vi "AssertControlInVisible_Tests.vi"(8 "error in":errorcluster) -> (0 "error out":errorcluster)   [LabVIEW 2016, in "DronaTest.lvlib"]
uses:
  DronaTest.lvlib
  APIs/Stimulus/ControlValue/ValueSignalByPathString.vi
  APIs/Assert/AssertControlProperty/AssertControlVisible/AssertInvisible.vi
  Drona.lvlib
  APIs/Stimulus/ControlValue/ControlValue.lvlib
  <vilib>/addons/_JKI Toolkits/Caraya/classes/Test/Test.lvclass
  APIs/Assert/AssertControlProperty/AssertControlVisible/AssertControlVisible.lvlib
  <vilib>/addons/_JKI Toolkits/Caraya/classes/Assert/Assert.lvclass
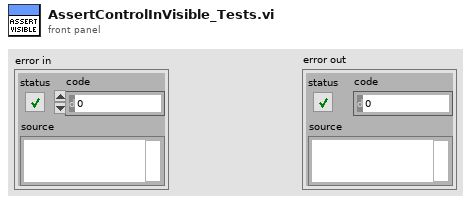
[diagram p1: front panel]
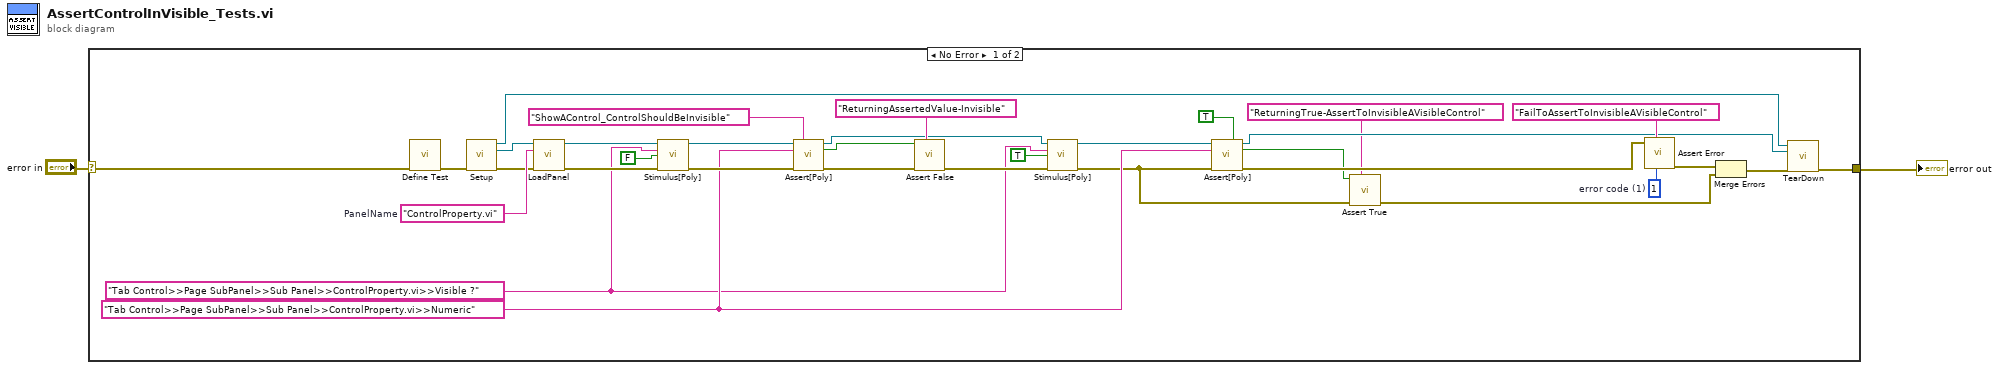
[diagram p0: block diagram]
diagram:
  n1 = case shown="No Error" "error in" {
    selector: "error in" -> [w35 w36]
    tunnel: [w25 w36] -> w1
    frame No Error {
      w13 = 1  # error code (1)
      w15 = "Tab Control>>Page SubPanel>>Sub Panel>>ControlProperty.vi>>Numeric" ("Control Path")
      w8 = "Tab Control>>Page SubPanel>>Sub Panel>>ControlProperty.vi>>Visible ?" ("Control Path")
      w34 = "ControlProperty.vi"  # PanelName
      n2 = call <vilib>:"Define Test.vi"("error in (no error)"=w35) -> ("error out"=w28:errorcluster)  [unwired: 9 in, 1 out]
      n3 = call "Setup.vi"("error in"=w28) -> ("Application Ref"=w24:refnum<vi>, "VI out"=w29:refnum<vi>, "error out"=w30:errorcluster)  [unwired: 12 in]
      n4 = call "LoadPanel.vi"("VI in"=w29, "Item Name"=w34, "error in"=w30) -> ("VI out"=w21:refnum<vi>, "error out"=w31:errorcluster)  [unwired: 11 in]
      n5 = call-poly "Stimulus[Poly].vi"("VI Reference In"=w21, "Control Path"=w8, "Value (Signaling)"=FALSE, "error in"=w31) -> ("VI Reference Out"=w33:refnum<vi>, "error out"=w23:errorcluster)  [unwired: 10 in]
      n6 = call-poly "Assert[Poly].vi"("VI Reference In"=w33, "Label"="ShowAControl_ControlShouldBeInvisible" ("string"), "Control Path"=w15, "Error In"=w23) -> ("VI Reference Out"=w10:refnum<vi>, "Asserted Value"=w22:bool, "Error Out"=w26:errorcluster)  [unwired: 9 in]
      n7 = call <vilib>:"Assert False.vi"("Label"="ReturningAssertedValue-Invisible", "error in (no error)"=w26, "False?"=w22) -> ("error out"=w11:errorcluster)  [unwired: 7 in, 1 out]
      n8 = call-poly "Stimulus[Poly].vi"("VI Reference In"=w10, "Control Path"=w8, "Value (Signaling)"=TRUE, "error in"=w11) -> ("VI Reference Out"=w9:refnum<vi>, "error out"=w7:errorcluster)  [unwired: 10 in]
      n9 = call-poly "Assert[Poly].vi"("VI Reference In"=w9, "Assert Only? (F)"=TRUE, "Control Path"=w15, "Error In"=w7) -> ("VI Reference Out"=w14:refnum<vi>, "Asserted Value"=w5:bool, "Error Out"=w19:errorcluster)  [unwired: 9 in]
      n10 = call <vilib>:"Assert True.vi"("Label"="ReturningTrue-AssertToInvisibleAVisibleControl", "error in (no error)"=w7, "True?"=w5) -> ("error out"=w3:errorcluster)  [unwired: 7 in, 1 out]
      n11 = call <vilib>:"Assert Error.vi"("error code (1)"=w13, "Label"="FailToAssertToInvisibleAVisibleControl", "Error?"=w19) -> ("error out"=w18:errorcluster)  [unwired: 7 in, 1 out]
      n12 = Merge Errors(w18, w3) -> (w4:errorcluster)
      n13 = call "TearDown.vi"("Application Ref"=w24, "VI in"=w14, "error in (no error)"=w4) -> ("error out"=w25:errorcluster)  [unwired: 12 in]
    }
    frame Error {
    }
  }
  "error out" <- w1
